vi "Get-PAQ-tags.vi"(8 "error in (no error)":errorcluster, 11 "HISW in":refnum<class "HISW.lvclass">) -> (0 "error out":errorcluster, 2 "PAQ_TAGs":string[](array[string]), 3 "HISW out":refnum<class "HISW.lvclass">)   [LabVIEW 2020, in "Sgraph_lib_V1.lvlib" / "HISW.lvclass"]
doc: "Read TAGs of Qtype : PAQ"
uses:
  HISW.lvclass
  C:/Sgraph/Sgraph/source/FAMM/FAMM.lvclass
  FAMM/FAMM.lvclass/FAMM.ctl
  FAMM/FAMM.lvclass
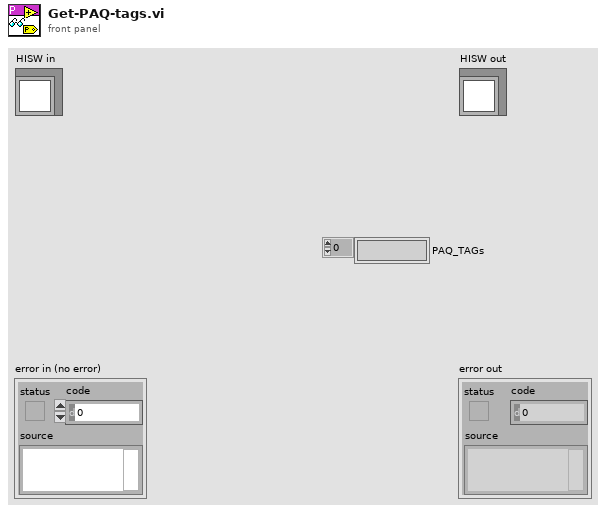
[diagram p1: front panel]
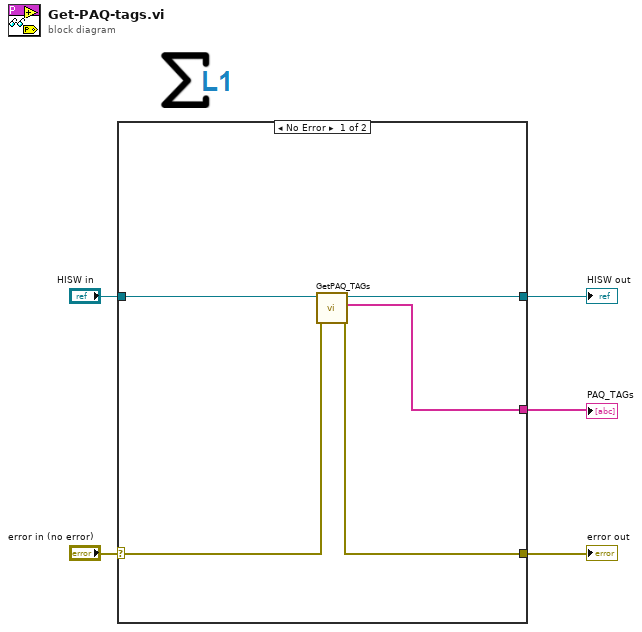
[diagram p0: block diagram]
diagram:
  n1 = case shown="No Error" "error in (no error)" {
    selector: "error in (no error)" -> [w8 w12]
    tunnel: [w10 w12] -> w4
    tunnel: [w7 w11] -> w2
    tunnel: "HISW in" -> [w6 w11]
    tunnel: [w9 _] -> w1
    frame No Error {
      n2 = call "GetPAQ_TAGs.vi"("error in (no error)"=w8, "FAMM in"=w6) -> ("error out"=w10:errorcluster, "PAQ_TAGs"=w9:string[], "FAMM out"=w7:refnum<class "HISW.lvclass">)  [unwired: 7 in]
    }
    frame Error {
    }
  }
  "error out" <- w4
  "HISW out" <- w2
  "PAQ_TAGs" <- w1
